vi "PathPlanner_ObstacleGrid_ToOccupancyGrid.vi"(11 "PathPlanner_Grid":T1) -> (0 "error out":errorcluster, 3 "map reference out":refnum<data-value>)   [LabVIEW 2019, in "PathPlanner24.lvlib"]
doc: "Converts a PathPlanner Obstacle Grid to a LabVIEW occumance map reference.\n\nInputs: \n - PathPlanner_ObstacleGrid - cluster -- data to convert\n\nOutputs:\n - Map Reference Out -- reference -- Reference to Occupancy map for use by LabVIEW AD* pathfinding.\n - Error out - cluster - Error cluster"
uses:
  PathPlanner24.lvlib
  TypeDef/PathPlannerObstacleGrid.ctl
  <vilib>/robotics/Navigation/shared/WorldMap/OccupancyGridWorldMap/NI_Robotics_OccupancyGridWorldMap.lvclass
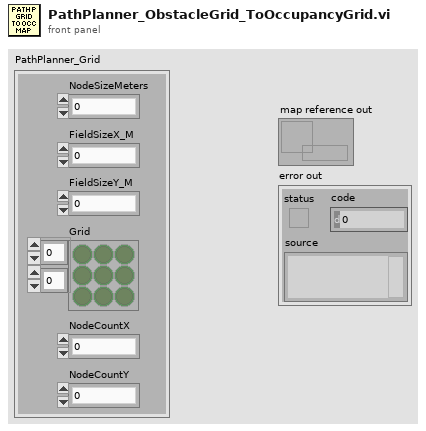
[diagram p1: front panel]
types:
  T1 = typedef "PathPlanner24.lvlib/PathPlannerObstacleGrid.ctl" = cluster{"NodeSizeMeters":dbl, "Grid":bool[][], "NodeCountX":i32, "NodeCountY":i32, "FieldSizeX_M":dbl, "FieldSizeY_M":dbl}
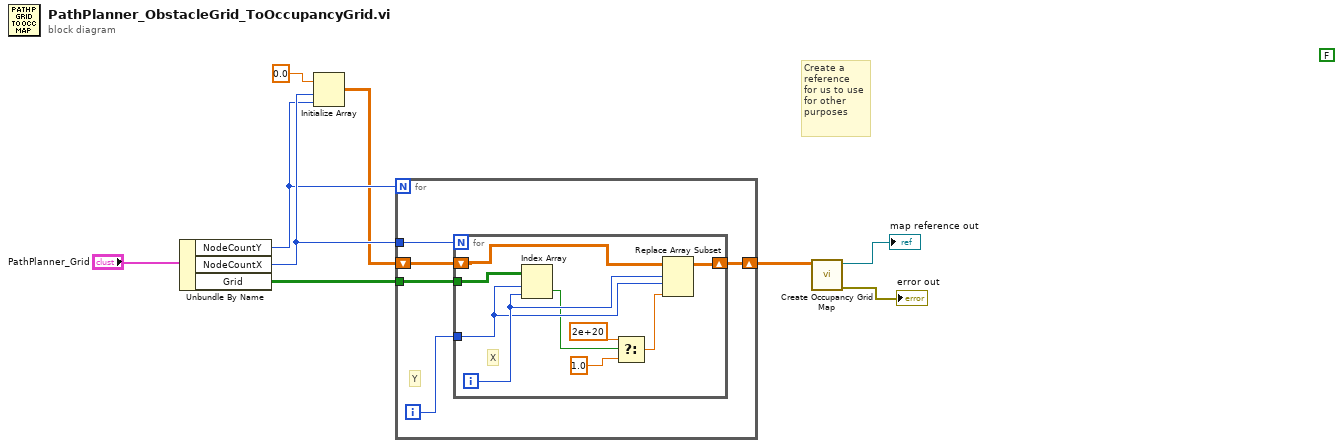
[diagram p0: block diagram]
diagram:
  (unwired) FALSE ("Error")
  # "Create a \nreference\nfor us to use\nfor other \npurposes"
  n1 = Unbundle By Name("PathPlanner_Grid") -> ("NodeCountY"=w4:i32, "NodeCountX"=w5:i32, "Grid"=w8:bool[][])
  n2 = Initialize Array(0.0 ("element"), w5, w4) -> (w2:dbl[][])
  n3 = for {
    N: w4 -> [_]
    tunnel: w8 -> [w14]
    tunnel: w5 -> [w13]
    shift-right: [w10] -> w1
    shift-left: w2 -> [w11]
    i -> [w12]
    # "Y"
    n4 = for {
      N: w13 -> [_]
      tunnel: w14 -> [w21]
      tunnel: w12 -> [w18]
      shift-right: [w15] -> w10
      shift-left: w11 -> [w20]
      i -> [w19]
      # "X"
      n5 = Index Array(array=w21, index (row)=w18, index (col)=w19) -> (element=w17:bool)
      n6 = Select(t=2e+20, s=w17, f=1.0) -> (s? t:f=w16:dbl)
      n7 = Replace Array Subset(array=w20, new element=w16, index (row)=w19, index (col)=w18) -> (w15:dbl[][])
    }
  }
  n8 = call <vilib>:"Create Occupancy Grid Map.vi"("occupancy grid"=w1) -> ("error out"=→"error out":errorcluster, "map reference out"=→"map reference out":refnum<data-value>)  [unwired: 9 in]
